vi "Advance Configurable Step.vi"(7 "checks passed":bool, 8 "popup acknowledged":bool, 9 "now ms":dbl, 10 "Step":T2, 11 "State":T1) -> (0 "retest":bool, 1 "failed":bool, 2 "send actions":bool, 3 "Next State":T1, 5 "retest step":i32)   [LabVIEW 2026]
doc: "Pure step phase logic. Phases: 0 pre-delay, 1 popup, 2 actions, 3 checks, 4 post-delay, 5 done, 6 failed. Anything not configured passes straight through. A popup that times out unanswered fails the step, and a popup timeout of 0 waits for the operator. On a check timeout the step retries once if retest is enabled, otherwise it fails. AF-free."
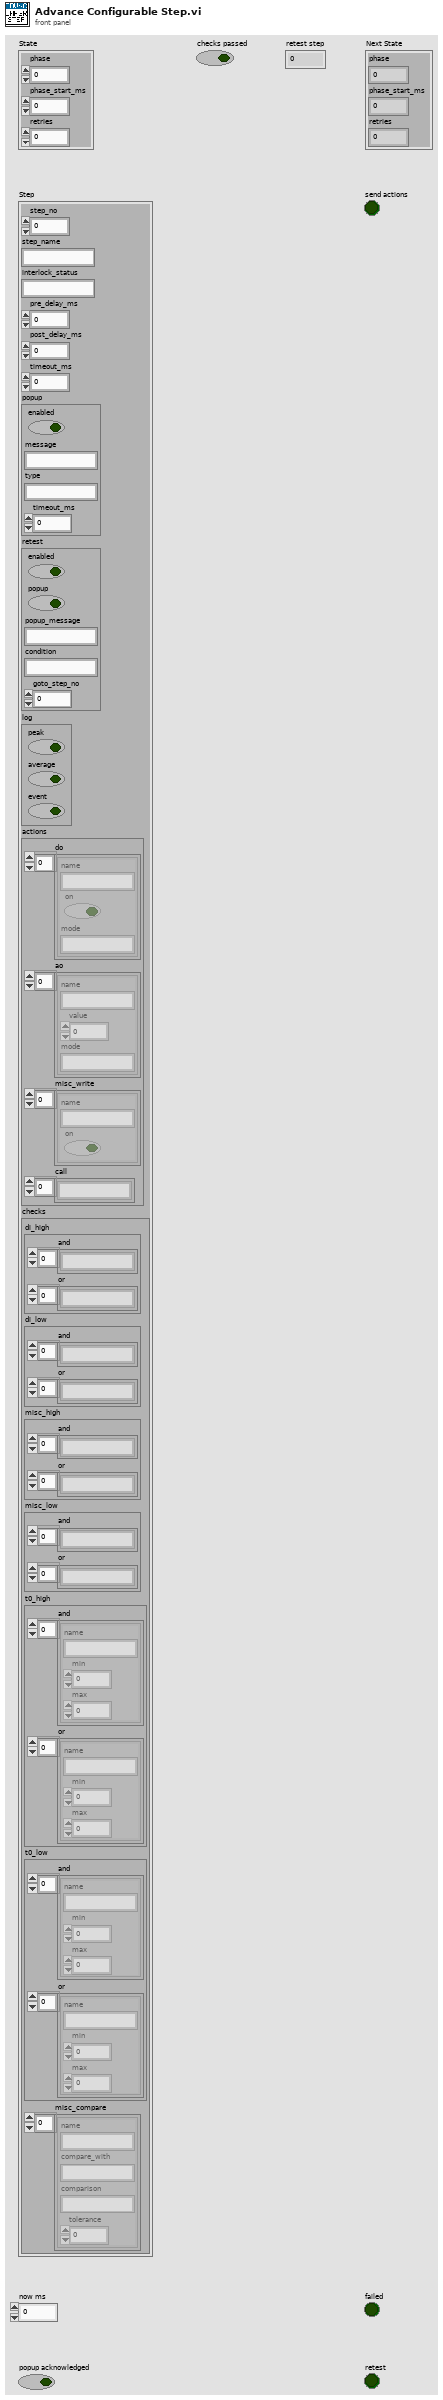
[diagram p1: front panel]
types:
  T1 = cluster{"phase":i32, "phase_start_ms":dbl, "retries":i32}
  T2 = cluster{"step_no":i32, "step_name":string, "interlock_status":string, "pre_delay_ms":dbl, "post_delay_ms":dbl, "timeout_ms":dbl, "popup":cluster{"enabled":bool, "message":string, "type":string, "timeout_ms":dbl}, "retest":cluster{"enabled":bool, "popup":bool, "popup_message":string, "condition":string, "goto_step_no":i32}, "log":cluster{"peak":bool, "average":bool, "event":bool}, "actions":cluster{"do":cluster{"name":string, "on":bool, "mode":string}[], "ao":cluster{"name":string, "value":dbl, "mode":string}[], "misc_write":cluster{"name":string, "on":bool}[], "call":string[]}, "checks":cluster{"di_high":cluster{"and":string[], "or":string[]}, "di_low":cluster{"and":string[], "or":string[]}, "misc_high":cluster{"and":string[], "or":string[]}, "misc_low":cluster{"and":string[], "or":string[]}, "t0_high":cluster{"and":cluster{"name":string, "min":dbl, "max":dbl}[], "or":cluster{"name":string, "min":dbl, "max":dbl}[]}, "t0_low":cluster{"and":cluster{"name":string, "min":dbl, "max":dbl}[], "or":cluster{"name":string, "min":dbl, "max":dbl}[]}, "misc_compare":cluster{"name":string, "compare_with":string, "comparison":string, "tolerance":dbl}[]}}
  T3 = cluster{"enabled":bool, "message":string, "type":string, "timeout_ms":dbl}
  T4 = cluster{"enabled":bool, "popup":bool, "popup_message":string, "condition":string, "goto_step_no":i32}
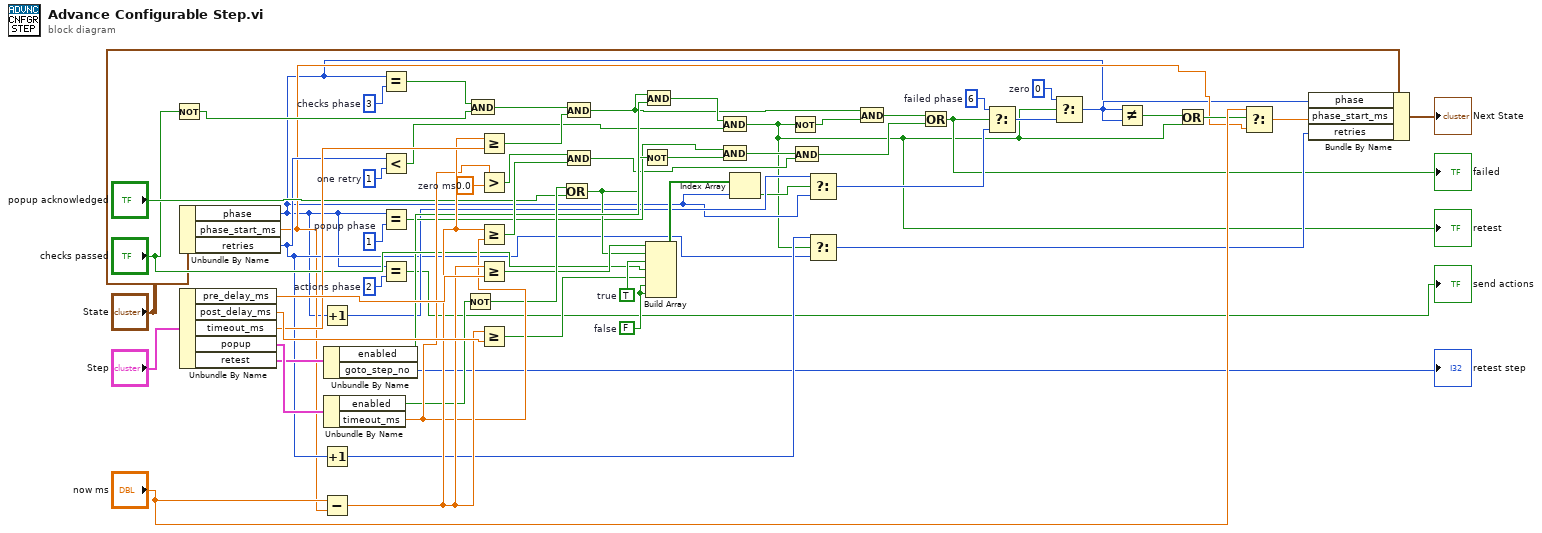
[diagram p0: block diagram]
diagram:
  w33 = 1  # popup phase
  w36 = 1  # one retry
  w21 = 6  # failed phase
  w6 = 2  # actions phase
  w43 = 3  # checks phase
  w45 = FALSE  # false
  w47 = TRUE  # true
  w19 = 0  # zero
  w56 = 0.0  # zero ms
  n1 = Not(x="checks passed") -> (.not. x?=w40:bool)
  n2 = Unbundle By Name("State") -> ("phase"=w7:i32, "phase_start_ms"=w12:dbl, "retries"=w16:i32)
  n3 = Unbundle By Name("Step") -> ("pre_delay_ms"=w59:dbl, "post_delay_ms"=w58:dbl, "timeout_ms"=w57:dbl, "popup"=w61:T3, "retest"=w60:T4)
  n4 = Increment(x=w7) -> (x+1=w23:i32)
  n5 = Increment(x=w16) -> (x+1=w17:i32)
  n6 = Subtract(x="now ms", y=w12) -> (x-y=w55:dbl)
  n7 = Unbundle By Name(w60) -> ("enabled"=w37:bool, "goto_step_no"=→"retest step":i32)
  n8 = Unbundle By Name(w61) -> ("enabled"=w51:bool, "timeout_ms"=w54:dbl)
  n9 = Equal?(x=w7, y=w43) -> (x = y?=w41:bool)
  n10 = Less?(x=w16, y=w36) -> (x < y?=w34:bool)
  n11 = Equal?(x=w7, y=w33) -> (x = y?=w31:bool)
  n12 = Equal?(x=w7, y=w6) -> (x = y?=→"send actions":bool)
  n13 = Not(x=w51) -> (.not. x?=w50:bool)
  n14 = And(x=w41, y=w40) -> (x .and. y?=w39:bool)
  n15 = Greater Or Equal?(x=w55, y=w57) -> (x >= y?=w38:bool)
  n16 = Greater?(x=w54, y=w56) -> (0:w53:bool)
  n17 = Greater Or Equal?(x=w55, y=w54) -> (x >= y?=w52:bool)
  n18 = Greater Or Equal?(x=w55, y=w59) -> (x >= y?=w48:bool)
  n19 = Greater Or Equal?(x=w55, y=w58) -> (x >= y?=w46:bool)
  n20 = Or(x=w50, y="popup acknowledged") -> (x .or. y?=w32:bool)
  n21 = And(x=w39, y=w38) -> (x .and. y?=w27:bool)
  n22 = And(x=w53, y=w52) -> (x .and. y?=w28:bool)
  n23 = Not(x=w32) -> (.not. x?=w30:bool)
  n24 = And(x=w27, y=w37) -> (x .and. y?=w35:bool)
  n25 = Build Array(w48, w32, w47, "checks passed", w46, w45, w45) -> (w44:bool[])
  n26 = And(x=w35, y=w34) -> (x .and. y?=w2:bool)
  "retest" <- w2
  n27 = And(x=w31, y=w30) -> (x .and. y?=w29:bool)
  n28 = Index Array(array=w44, index=w7) -> (element=w22:bool)
  n29 = Not(x=w2) -> (.not. x?=w26:bool)
  n30 = And(x=w29, y=w28) -> (x .and. y?=w24:bool)
  n31 = Select(t=w23, s=w22, f=w7) -> (s? t:f=w20:i32)
  n32 = Select(t=w17, s=w2, f=w16) -> (s? t:f=w9:i32)
  n33 = And(x=w27, y=w26) -> (x .and. y?=w25:bool)
  n34 = Or(x=w25, y=w24) -> (x .or. y?=w3:bool)
  "failed" <- w3
  n35 = Select(t=w21, s=w3, f=w20) -> (s? t:f=w18:i32)
  n36 = Select(t=w19, s=w2, f=w18) -> (s? t:f=w11:i32)
  n37 = Not Equal?(x=w11, y=w7) -> (x != y?=w15:bool)
  n38 = Or(x=w15, y=w2) -> (x .or. y?=w13:bool)
  n39 = Select(t="now ms", s=w13, f=w12) -> (s? t:f=w10:dbl)
  n40 = Bundle By Name(cluster="State", "phase"=w11, "phase_start_ms"=w10, "retries"=w9) -> (→"Next State":T1)
